vi "CANsub_API_Loopback_Example.vi"() -> ()   [LabVIEW 2021]
doc: "CANsub API loopback example (CH1–CH2 cable): sends a numbered frame on tx channel every period (Write_Frame), receives it on rx channel (Read, Frame_Get), checks the sequence and measures the host round trip; drains the TX acks on tx channel. Two CANsub_Channel objects, one per channel. Uses only CANsub_API.lvlib."
uses:
  api/CANsub_Channel/CANsub_Channel.lvclass
  Example_Loopback_Stats.ctl
  common/Typedefs/CANsub_connection.ctl
  common/CANsub_Common.lvlib
  common/Typedefs/CANsub_Bit_Rates.ctl
  api/Typedefs/CANsub_Filter.ctl
  api/CANsub_API.lvlib
  api/Typedefs/CANsub_Read_Mode.ctl
  api/Typedefs/CANsub_Ownership.ctl
  api/Typedefs/CANsub_Config.ctl
  api/Typedefs/CANsub_State.ctl
  common/Typedefs/Bit_Timing.ctl
  api/Typedefs/CANsub_Status.ctl
panel:
  out "error out":errorcluster
  out "status rx":T1
  out "status tx":T1
  out "received frames":string[][](table)
  out "stats":T4
  in  "stop":bool
  in  "max rows":i32=50
  in  "period ms":u32=10
  in  "tx id":u32=801 format="%.0x"
  in  "rx channel":u8=2
  in  "tx channel":u8=1
  in  "config":T5={"connection"={"host"="192.168.0.49", "channel"=2, "cert path"=path "/home/lvuser/cansub_root_cert.crt"}, "bit rates"={"nominal bit rate"=500000, "nominal sample point"=80.0, "data bit rate"=2000000, "data sample point"=80.0}, "listen only"=FALSE, "filters"=[], "read mode"=enum."Poll", "max bytes per read"=4096, "reader FIFO depth"=0, "reader priority"=0, "ownership"=enum."Direct"} {"filters"."f2" format="%.0x"; "filters"."f1" format="%.0x"}
  # "Needs CH1–CH2 cable; stop the harness and webCAN first. Run ? frames go out on tx channel every period, come back on rx channel. missing must stay 0; rtt = host round trip (send ? Read returns it). Stop closes both channels."
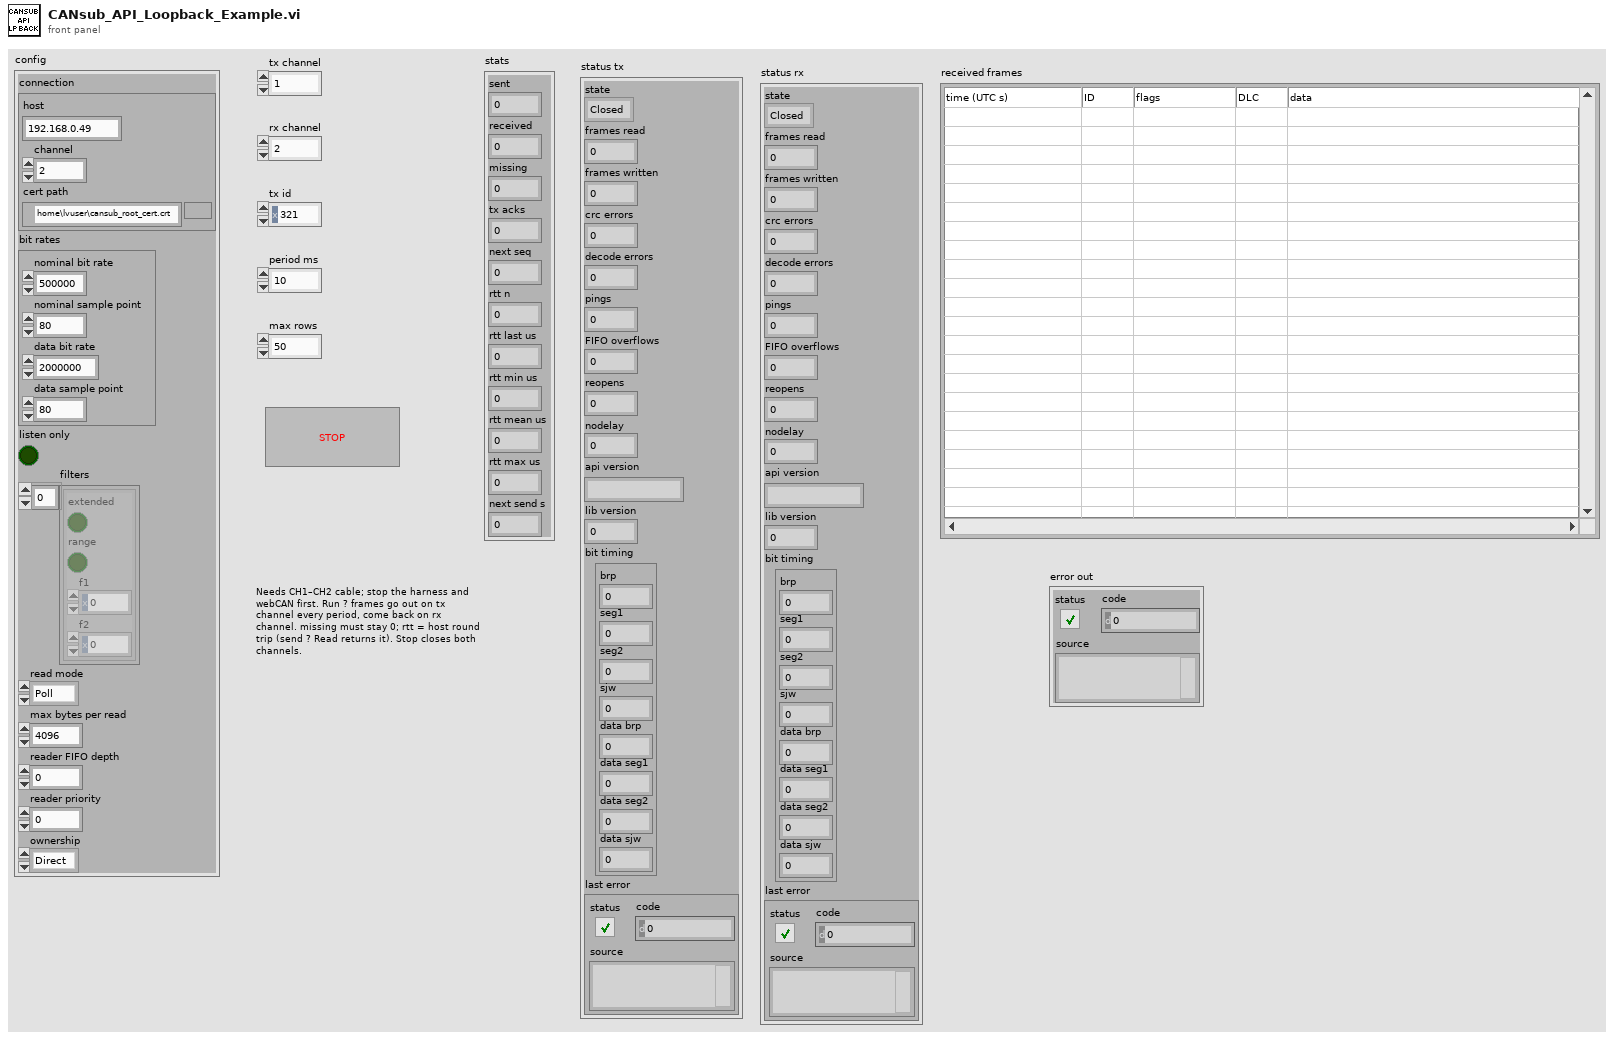
[diagram p1: front panel]
types:
  T1 = typedef "CANsub_API.lvlib/CANsub_Status.ctl" = cluster{"state":T2, "frames read":u32, "frames written":u32, "crc errors":u32, "decode errors":i32, "pings":u32, "FIFO overflows":u32, "reopens":u32, "nodelay":i32, "api version":string, "lib version":u32, "bit timing":T3, "last error":errorcluster}
  T2 = typedef "CANsub_API.lvlib/CANsub_State.ctl" = enum16{"Closed", "Open", "Lost"}
  T3 = typedef "CANsub_Common.lvlib/Bit_Timing.ctl" = cluster{"brp":u16, "seg1":u16, "seg2":u16, "sjw":u16, "data brp":u16, "data seg1":u16, "data seg2":u16, "data sjw":u16}
  T4 = typedef "Example_Loopback_Stats.ctl" = cluster{"sent":u32, "received":u32, "missing":u32, "tx acks":u32, "next seq":u32, "rtt n":u32, "rtt last us":dbl, "rtt min us":dbl, "rtt mean us":dbl, "rtt max us":dbl, "rtt sum us":dbl, "next send s":dbl, "send times":dbl[]}
  T5 = typedef "CANsub_API.lvlib/CANsub_Config.ctl" = cluster{"connection":T6, "bit rates":T7, "listen only":bool, "filters":T8[], "read mode":T9, "max bytes per read":i32, "reader FIFO depth":i32, "reader priority":i32, "ownership":T10}
  T6 = typedef "CANsub_Common.lvlib/CANsub_connection.ctl" = cluster{"host":string, "channel":u8, "cert path":path}
  T7 = typedef "CANsub_Common.lvlib/CANsub_Bit_Rates.ctl" = cluster{"nominal bit rate":u32, "nominal sample point":dbl, "data bit rate":u32, "data sample point":dbl}
  T8 = typedef "CANsub_API.lvlib/CANsub_Filter.ctl" = cluster{"extended":bool, "range":bool, "f1":u32, "f2":u32}
  T9 = typedef "CANsub_API.lvlib/CANsub_Read_Mode.ctl" = enum16{"Poll", "Reader"}
  T10 = typedef "CANsub_API.lvlib/CANsub_Ownership.ctl" = enum16{"Direct", "Shared"}
  T11 = typedef "CANsub_API.lvlib/CANsub_Frames.ctl" = cluster{"count":i32, "t_dev":dbl[], "id":u32[], "flags":u16[], "dlc":u8[], "data len":u8[], "data":u8[]}
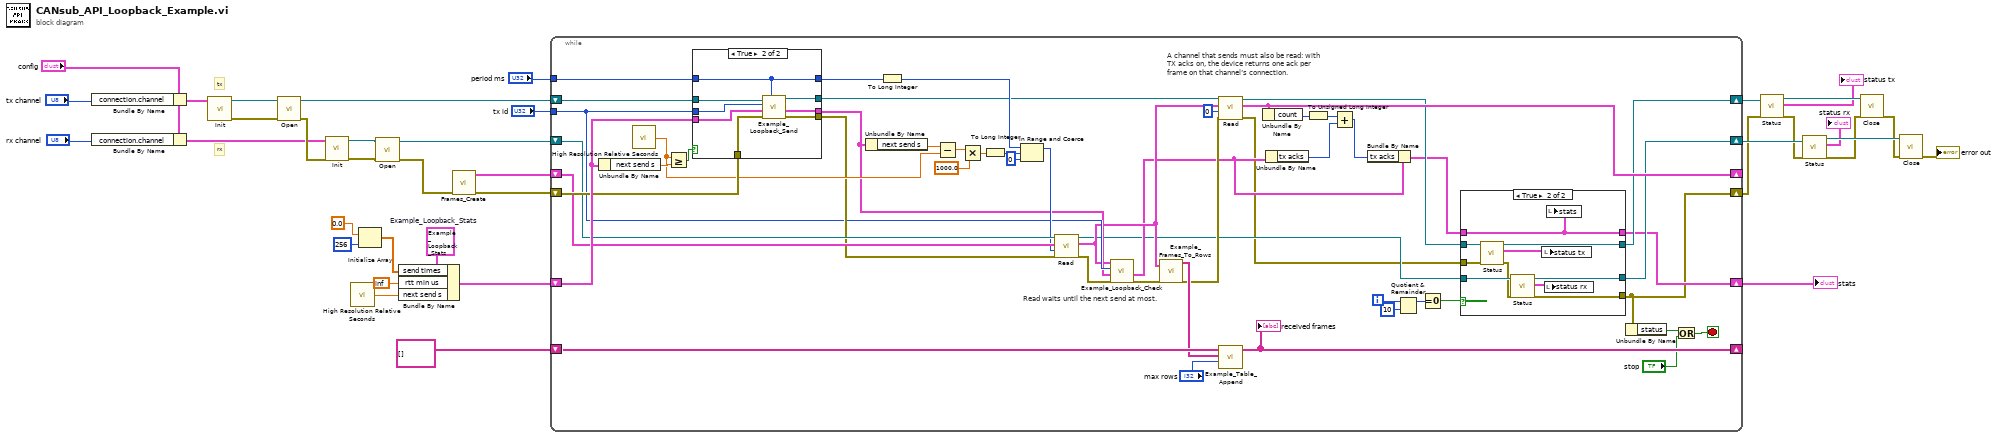
[diagram p0: block diagram]
diagram:
  w37 = T4 {"sent"=0, "received"=0, "missing"=0, "tx acks"=0, "next seq"=0, "rtt n"=0, "rtt last us"=0.0, "rtt min us"=0.0, "rtt mean us"=0.0, "rtt max us"=0.0, "rtt sum us"=0.0, "next send s"=0.0, "send times"=[]}  # Example_Loopback_Stats
  # "rx"
  # "tx"
  n1 = Bundle By Name(cluster="config", "connection.channel"="tx channel") -> (w22:T5)
  n2 = Bundle By Name(cluster="config", "connection.channel"="rx channel") -> (w21:T5)
  n3 = call "Init.vi"("config"=w22) -> ("error out"=w30:errorcluster, "channel out"=w31:refnum<class "CANsub_Channel.lvclass">)  [unwired: 8 in, 1 out]
  n4 = call-dynamic "Open.vi"("error in (no error)"=w30, "channel in"=w31) -> ("error out"=w29:errorcluster, "channel out"=w19:refnum<class "CANsub_Channel.lvclass">)  [unwired: 8 in]
  n5 = call "Init.vi"("error in (no error)"=w29, "config"=w21) -> ("error out"=w27:errorcluster, "channel out"=w28:refnum<class "CANsub_Channel.lvclass">)  [unwired: 7 in, 1 out]
  n6 = call <vilib>:"High Resolution Relative Seconds.vi"() -> ("relative seconds"=w36:dbl)
  n7 = Initialize Array(0.0 ("element"), 256 ("dimension size")) -> (w32:dbl[])
  n8 = call-dynamic "Open.vi"("error in (no error)"=w27, "channel in"=w28) -> ("error out"=w26:errorcluster, "channel out"=w18:refnum<class "CANsub_Channel.lvclass">)  [unwired: 8 in]
  n9 = Bundle By Name(cluster=w37, "send times"=w32, "rtt min us"=inf, "next send s"=w36) -> (w17:T4)
  n10 = call "Frames_Create.vi"("error in (no error)"=w26) -> ("error out"=w15:errorcluster, "frames"=w20:T11)  [unwired: 9 in]
  n11 = while {
    shift-right: [w53] -> _
    shift-left: w20 -> [w71]
    shift-right: [w45] -> w14
    shift-left: w19 -> [w86]
    shift-right: [w44] -> w12
    shift-left: w18 -> [w72]
    shift-right: [w42] -> w1
    shift-left: w17 -> [w84]
    shift-right: [w89] -> _
    shift-left: string[][] [] -> [w64]
    shift-right: [w38] -> w8
    shift-left: w15 -> [w82]
    tunnel: "tx id" -> [w68]
    tunnel: "period ms" -> [w85]
    i -> [w52]
    stop <- w39 stop-if-true
    # "A channel that sends must also be read: with TX acks on, the device returns one ack per frame on that channel’s connection."
    # "Read waits until the next send at most."
    n12 = Unbundle By Name(w84) -> ("next send s"=w87:dbl)
    n13 = call <vilib>:"High Resolution Relative Seconds.vi"() -> ("relative seconds"=w80:dbl)
    n14 = Greater Or Equal?(x=w80, y=w87) -> (x >= y?=w88:bool)
    n15 = case shown="True" w88 {
      tunnel: [w106 w114] -> w62
      tunnel: w86 -> [w106 w115]
      tunnel: w68 -> [_ w113]
      tunnel: w85 -> [w104 w108]
      tunnel: w84 -> [w107 w112]
      tunnel: [w107 w111] -> w67
      tunnel: w82 -> [w105 w110]
      tunnel: [w105 w109] -> w69
      tunnel: [w104 w108] -> w74
      frame False {
      }
      frame True {
        n16 = call "Example_Loopback_Send.vi"("period"=w108, "error in (no error)"=w110, "stats in"=w112, "tx id"=w113, "channel in"=w115) -> ("error out"=w109:errorcluster, "stats out"=w111:T4, "channel out"=w114:refnum<class "CANsub_Channel.lvclass">)  [unwired: 4 in]
      }
    }
    n17 = Unbundle By Name(w67) -> ("next send s"=w81:dbl)
    n18 = To Long Integer(number=w74) -> (32bit integer=w73:i32)
    n19 = Subtract(x=w81, y=w80) -> (x-y=w79:dbl)
    n20 = Multiply(x=w79, y=1000.0) -> (x*y=w77:dbl)
    n21 = To Long Integer(number=w77) -> (32bit integer=w76:i32)
    n22 = In Range and Coerce(upper limit=w73, x=w76, lower limit=0) -> (coerced(x)=w70:i32)  [unwired: 1 out]
    n23 = call-dynamic "Read.vi"("error in (no error)"=w69, "timeout ms"=w70, "frames in"=w71, "channel in"=w72) -> ("error out"=w66:errorcluster, "frames out"=w61:T11, "channel out"=w47:refnum<class "CANsub_Channel.lvclass">)  [unwired: 5 in]
    n24 = call "Example_Loopback_Check.vi"("error in (no error)"=w66, "stats in"=w67, "tx id"=w68, "frames"=w61) -> ("error out"=w65:errorcluster, "stats out"=w58:T4)  [unwired: 6 in]
    n25 = call "Example_Frames_To_Rows.vi"("error in (no error)"=w65, "frames"=w61) -> ("error out"=w59:errorcluster, "rows"=w63:string[][])  [unwired: 8 in]
    n26 = call-dynamic "Read.vi"("error in (no error)"=w59, "timeout ms"=0, "frames in"=w61, "channel in"=w62) -> ("error out"=w46:errorcluster, "frames out"=w53:T11, "channel out"=w48:refnum<class "CANsub_Channel.lvclass">)  [unwired: 5 in]
    n27 = call "Example_Table_Append.vi"("max rows"="max rows", "rows"=w63, "table in"=w64) -> ("table out"=w89:string[][])  [unwired: 8 in]
    "received frames" <- w89
    n28 = Unbundle By Name(w53) -> ("count"=w57:i32)
    n29 = Unbundle By Name(w58) -> ("tx acks"=w55:u32)
    n30 = To Unsigned Long Integer(number=w57) -> (unsigned 32bit integer=w56:u32)
    n31 = Add(x=w56, y=w55) -> (x+y=w54:u32)
    n32 = Bundle By Name(cluster=w58, "tx acks"=w54) -> (w43:T4)
    n33 = Quotient & Remainder(x=w52, y=10) -> (x-y*floor(x/y)=w50:i32)  [unwired: 1 out]
    n34 = Equal To 0?(x=w50) -> (x = 0?=w49:bool)
    n35 = case shown="True" w49 {
      tunnel: w48 -> [w93 w103]
      tunnel: w47 -> [w92 w102]
      tunnel: [w93 w101] -> w45
      tunnel: [w92 w100] -> w44
      tunnel: w46 -> [w91 w99]
      tunnel: [w91 w95] -> w38
      tunnel: w43 -> [w90 w94]
      tunnel: [w90 w94] -> w42
      frame False {
      }
      frame True {
        n36 = call-dynamic "Status.vi"("error in (no error)"=w99, "channel in"=w103) -> ("error out"=w97:errorcluster, "status"=w98:T1, "channel out"=w101:refnum<class "CANsub_Channel.lvclass">)  [unwired: 7 in]
        n37 = call-dynamic "Status.vi"("error in (no error)"=w97, "channel in"=w102) -> ("error out"=w95:errorcluster, "status"=w96:T1, "channel out"=w100:refnum<class "CANsub_Channel.lvclass">)  [unwired: 7 in]
        n38 = local write "status tx"(w98) -> ()
        n39 = local write "status rx"(w96) -> ()
        n40 = local write "stats"(w94) -> ()
      }
    }
    n41 = Unbundle By Name(w38) -> ("status"=w41:bool)
    n42 = Or(x=w41, y="stop") -> (x .or. y?=w39:bool)
  }
  "stats" <- w1
  n43 = call-dynamic "Status.vi"("error in (no error)"=w8, "channel in"=w14) -> ("error out"=w7:errorcluster, "status"=→"status tx":T1, "channel out"=w13:refnum<class "CANsub_Channel.lvclass">)  [unwired: 7 in]
  n44 = call-dynamic "Status.vi"("error in (no error)"=w7, "channel in"=w12) -> ("error out"=w6:errorcluster, "status"=→"status rx":T1, "channel out"=w11:refnum<class "CANsub_Channel.lvclass">)  [unwired: 7 in]
  n45 = call-dynamic "Close.vi"("error in (no error)"=w6, "channel in"=w13) -> ("error out"=w5:errorcluster)  [unwired: 8 in, 1 out]
  n46 = call-dynamic "Close.vi"("error in (no error)"=w5, "channel in"=w11) -> ("error out"=→"error out":errorcluster)  [unwired: 8 in, 1 out]
